vi "Map to Tree.vi"(7 "Value Format":string, 10 "Tree":refnum<vi>, 11 "Map in":map{string[], T1}(c390)) -> ()   [LabVIEW 2020, in "VolatusDAQGenericGUI.lvlib"]
uses:
  VolatusDAQGenericGUI.lvlib
  AI Tree Entry.ctl
  Channel Entry.ctl
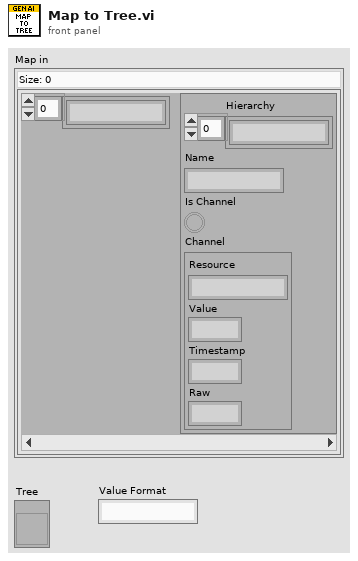
[diagram p1: front panel]
types:
  T1 = typedef "VolatusDAQGenericGUI.lvlib/AI Tree Entry.ctl" = cluster{"Hierarchy":string[], "Name":string, "Is Channel":bool, "Channel":T2}
  T2 = typedef "VolatusDAQGenericGUI.lvlib/Channel Entry.ctl" = cluster{"Resource":string, "Value":dbl, "Timestamp":dbl, "Raw":dbl}
  T3 = typedef "LVNodeAndColumnTypeDef.ctl" = cluster{"Node":string, "Column":i32}
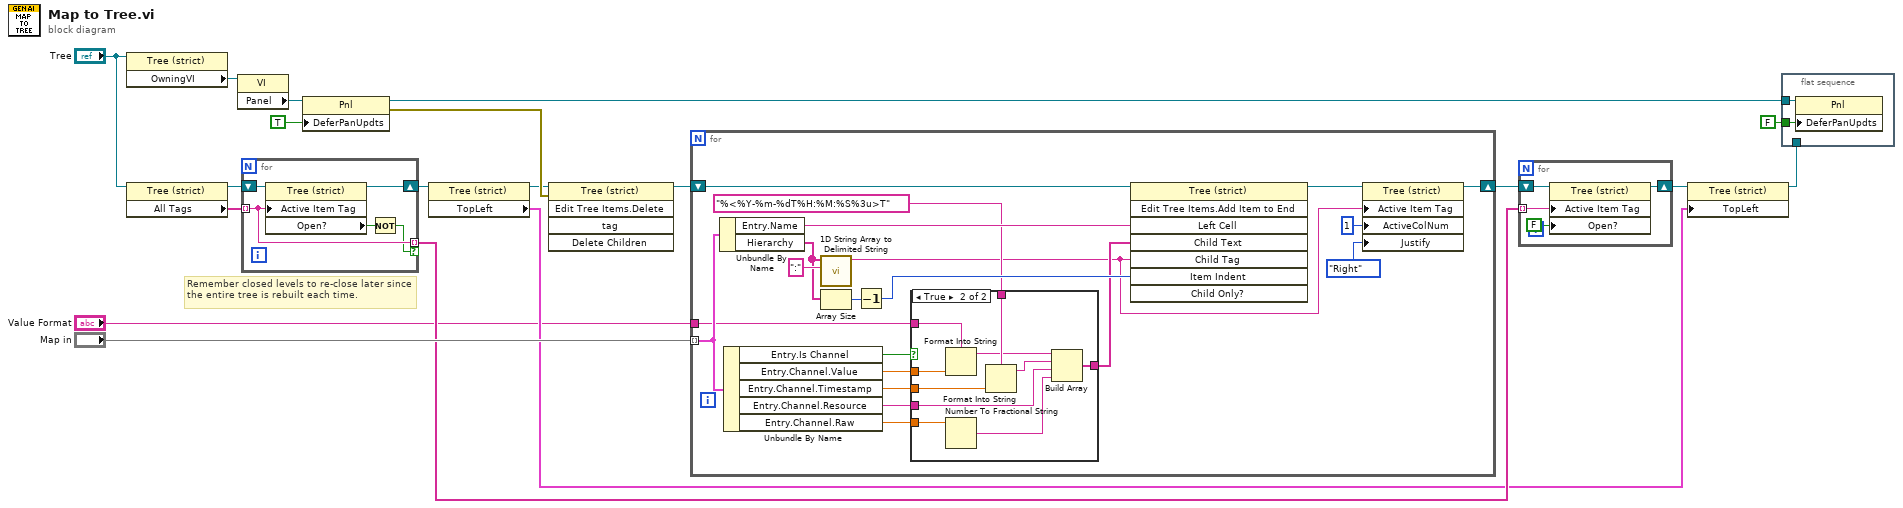
[diagram p0: block diagram]
diagram:
  # "Remember closed levels to re-close later since the entire tree is rebuilt each time."
  n1 = property class="Tree (strict)"(reference="Tree") -> ("OwningVI"=w18:refnum<vi>)  [unwired: 1 in, 2 out]
  n2 = property class="Tree (strict)"(reference="Tree") -> (reference out=w14:refnum<vi>, "All Tags"=w13:string[])  [unwired: 1 in, 1 out]
  n3 = property class="VI"(reference=w18) -> ("Panel"=w17:refnum<vi>)  [unwired: 1 in, 2 out]
  n4 = for {
    shift-right: [w20] -> w12
    shift-left: w14 -> [w24]
    tunnel: w13 -> [w22] mode=indexing
    tunnel: [w22] -> w6 mode=indexing if=w21
    n5 = property class="Tree (strict)"(reference=w24, "Active Item Tag"=w22) -> (reference out=w20:refnum<vi>, "Open?"=w23:bool)  [unwired: 1 in, 1 out]
    n6 = Not(x=w23) -> (.not. x?=w21:bool)
  }
  n7 = property class="Pnl"(reference=w17, "DeferPanUpdts"=TRUE ("Defer Panel Updates")) -> (reference out=w3:refnum<vi>, error out=w19:errorcluster)  [unwired: 1 in]
  n8 = property class="Tree (strict)"(reference=w12) -> (reference out=w11:refnum<vi>, "TopLeft"=w5:T3)  [unwired: 1 in, 1 out]
  n9 = invoke class="Tree (strict)" method="Edit Tree Items.Delete"(reference=w11, error in=w19) -> (reference out=w10:refnum<vi>)  [unwired: 3 in, 4 out]
  n10 = for {
    shift-right: [w26] -> w7
    shift-left: w10 -> [w44]
    tunnel: "Map in" -> [w38] mode=indexing
    tunnel: "Value Format" -> [w25]
    n11 = Unbundle By Name(w38) -> ("Entry.Name"=w43:string, "Hierarchy"=w41:string[])
    n12 = Unbundle By Name(w38) -> ("Entry.Is Channel"=w31:bool, "Entry.Channel.Value"=w37:dbl, "Entry.Channel.Timestamp"=w35:dbl, "Entry.Channel.Resource"=w34:string, "Entry.Channel.Raw"=w33:dbl)
    n13 = call <vilib>:"1D String Array to Delimited String.vi"("delimiter"=":", "string array"=w41) -> ("delimited string"=w29:string)  [unwired: 9 in]
    n14 = Array Size(array=w41) -> (size(s)=w40:i32)
    n15 = Decrement(x=w40) -> (x-1=w39:i32)
    n16 = case shown="True" w31 {
      tunnel: w37 -> [_ w46]
      tunnel: "%<%Y-%m-%dT%H:%M:%S%3u>T" -> [_ w54]
      tunnel: w35 -> [_ w53]
      tunnel: w34 -> [_ w51]
      tunnel: w33 -> [_ w50]
      tunnel: [_ w48] -> w32
      tunnel: w25 -> [_ w45]
      frame False {
      }
      frame True {
        n17 = Format Into String(format string=w45, w46) -> (resulting string=w47:string)  [unwired: 2 in, 1 out]
        n18 = Number To Fractional String(number=w50) -> (F-format string=w49:string)  [unwired: 3 in]
        n19 = Format Into String(format string=w54, w53) -> (resulting string=w52:string)  [unwired: 2 in, 1 out]
        n20 = Build Array(w47, w52, w51, w49) -> (w48:string[])
      }
    }
    n21 = invoke class="Tree (strict)" method="Edit Tree Items.Add Item to End"(reference=w44, "Left Cell"=w43, "Child Text"=w32, "Child Tag"=w29, "Item Indent"=w39) -> (reference out=w30:refnum<vi>)  [unwired: 3 in, 7 out]
    n22 = property class="Tree (strict)"(reference=w30, "Active Item Tag"=w29, "ActiveColNum"=1 ("Active Cell:Active Column Number"), "Justify"=enum16{"Left", "Center", "Right"}."Right" ("Active Cell:Cell Justification")) -> (reference out=w26:refnum<vi>)  [unwired: 1 in, 1 out]
  }
  n23 = for {
    shift-right: [w57] -> w8
    shift-left: w7 -> [w58]
    tunnel: w6 -> [w55] mode=indexing
    n24 = property class="Tree (strict)"(reference=w58, "Active Item Tag"=w55, "Open?"=FALSE ("Active Item:Open?")) -> (reference out=w57:refnum<vi>)  [unwired: 1 in, 1 out]
  }
  n25 = property class="Tree (strict)"(reference=w8, "TopLeft"=w5) -> (reference out=w2:refnum<vi>)  [unwired: 1 in, 1 out]
  n26 = flat-sequence {
    tunnel: FALSE ("Defer Panel Updates") -> [w60]
    tunnel: w3 -> [w59]
    tunnel: w2 -> [_]
    frame #0 {
      n27 = property class="Pnl"(reference=w59, "DeferPanUpdts"=w60) -> ()  [unwired: 1 in, 2 out]
    }
  }
